vi "Create.vi"(8 "error in (no error)":errorcluster, 9 "HTTP Manager":refnum<class "MessageQ.lvclass">, 10 "VolatusAPI":refnum<class "VolatusAPI.lvclass">) -> (0 "error out":errorcluster, 3 "VolatusVariableResolver out":refnum<class "VolatusVariableResolver.lvclass">)   [LabVIEW 2020, in "Volatus.lvlib" / "VolatusVariableResolver.lvclass"]
uses:
  VolatusVariableResolver.lvclass
  VolatusAPI/VolatusAPI.lvclass
  MessageQ/MessageQ.lvclass
  VolatusVariableResolver.lvclass/VolatusVariableResolver.ctl
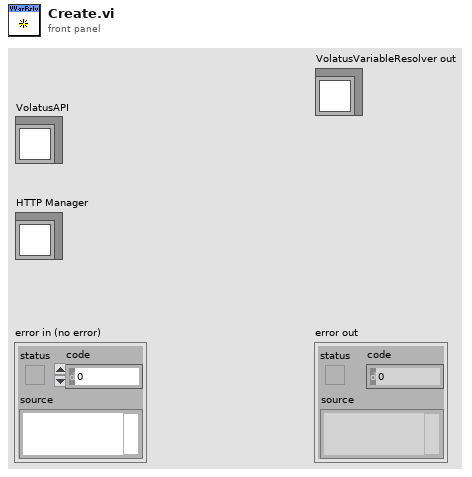
[diagram p1: front panel]
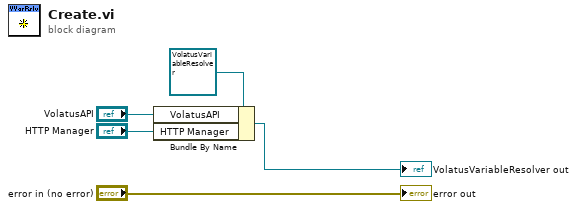
[diagram p0: block diagram]
diagram:
  n1 = Bundle By Name(cluster=refnum<class "VolatusVariableResolver.lvclass"> refnum ("VolatusVariableResolver in"), "VolatusAPI"="VolatusAPI", "HTTP Manager"="HTTP Manager") -> (→"VolatusVariableResolver out":refnum<class "VolatusVariableResolver.lvclass">)
  "error out" <- "error in (no error)"
